vi "ChopperTEST.vi"() -> ()   [LabVIEW 2013]
uses:
  <vilib>/DAQmx/configure/timing.llb/DAQmx Timing (Sample Clock).vi
  <vilib>/DAQmx/write.llb/DAQmx Write (Digital Wfm 1Chan NSamp).vi
  <vilib>/Analysis/NI_AALBase.lvlib
  <vilib>/Analysis/1siggen.llb/Ramp Pattern by Samples.vi
  <vilib>/DAQmx/write.llb/DAQmx Write (Analog 1D Wfm NChan NSamp).vi
  <resource>/objmgr/daqmx.rc
  <vilib>/DAQmx/create/channels.llb/DAQmx Create Channel (CO-Pulse Generation-Frequency).vi
  <vilib>/DAQmx/configure/timing.llb/DAQmx Timing (Implicit).vi
  <vilib>/Waveform/DWDTOps.llb/DWDT Boolean Array to Digital.vi
  <vilib>/DAQmx/create/channels.llb/DAQmx Create Channel (AO-Voltage-Basic).vi
  <vilib>/DAQmx/create/channels.llb/DAQmx Create Channel (DO-Digital Output).vi
panel:
  in  "Source_GATE_DutyCicle (%)":dbl(slide)=4.0000000000000036 min=0.1 max=99.9 step=0.1 scale=0.0..100.0
  in  "Source_GATE_period (ms)":dbl(slide)=60.0 scale=0.0..1000.0
  out "Faraday IN 2":bool
  in  "Faraday IN":bool
  in  "Chopper ON":bool=TRUE
  out "Chopper ON 2":bool=TRUE
  in  "Vmon_L (us)":i32(slide)=920 scale=0.0..3000.0
  in  "Vmon_H (us)":i32(slide)=27 scale=0.0..1000.0
  in  "Vmon_R (us)":i32(slide)=7 scale=0.0..40.0
  in  "Vmon_min (V)":dbl=-4.0 format="%#_13g"
  in  "Vmon_max (V)":dbl format="%#_13g"
  in  "Vmon_F (us)":i32(slide)=8 scale=0.0..40.0
  in  "ACCT_F (us)":i32(slide)=10 scale=0.0..40.0
  in  "ACCT_max (V)":dbl=1.0 format="%#_13g"
  in  "ACCT_min (V)":dbl=-1.0 format="%#_13g"
  in  "ACCT_R (us)":i32(slide)=9 scale=0.0..40.0
  in  "ACCT_H (us)":i32(slide)=20 scale=0.0..1000.0
  in  "ACCT_L (us)":i32(slide)=920 scale=0.0..3000.0
  in  "CH_GATE_H (us)":i32(slide)=34 scale=0.0..100.0
  in  "CH_GATE_L (us)":i32(slide)=920 scale=0.0..3000.0
  in  "Stop Button":bool
  # "Chopper GATE (pins 65,82)"
  # "Vmon AO0 (pins 15,16)"
  # "Source GATE (pins 89,82)"
  # "ACCT AO1 (pins 31,32)"
  # "Faraday IN (pins 67,82)"
  # "Chopper ON (pins 68,82)"
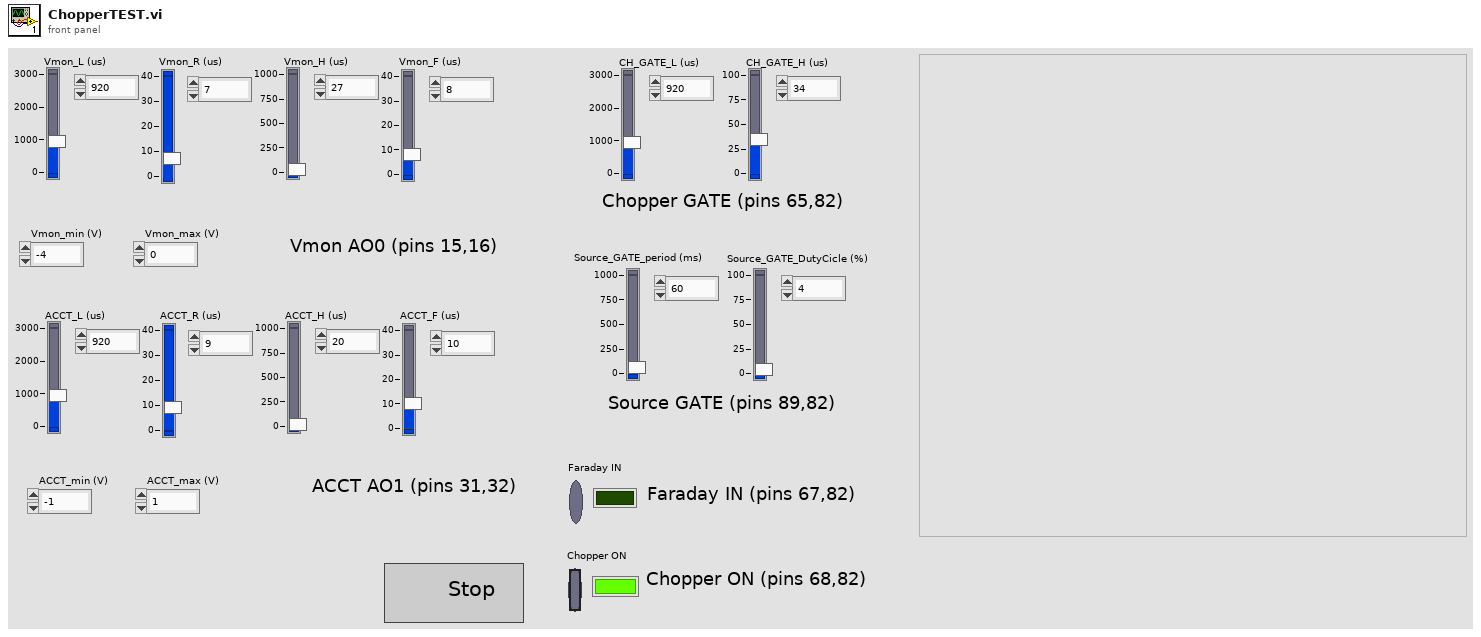
[diagram p1: front panel]
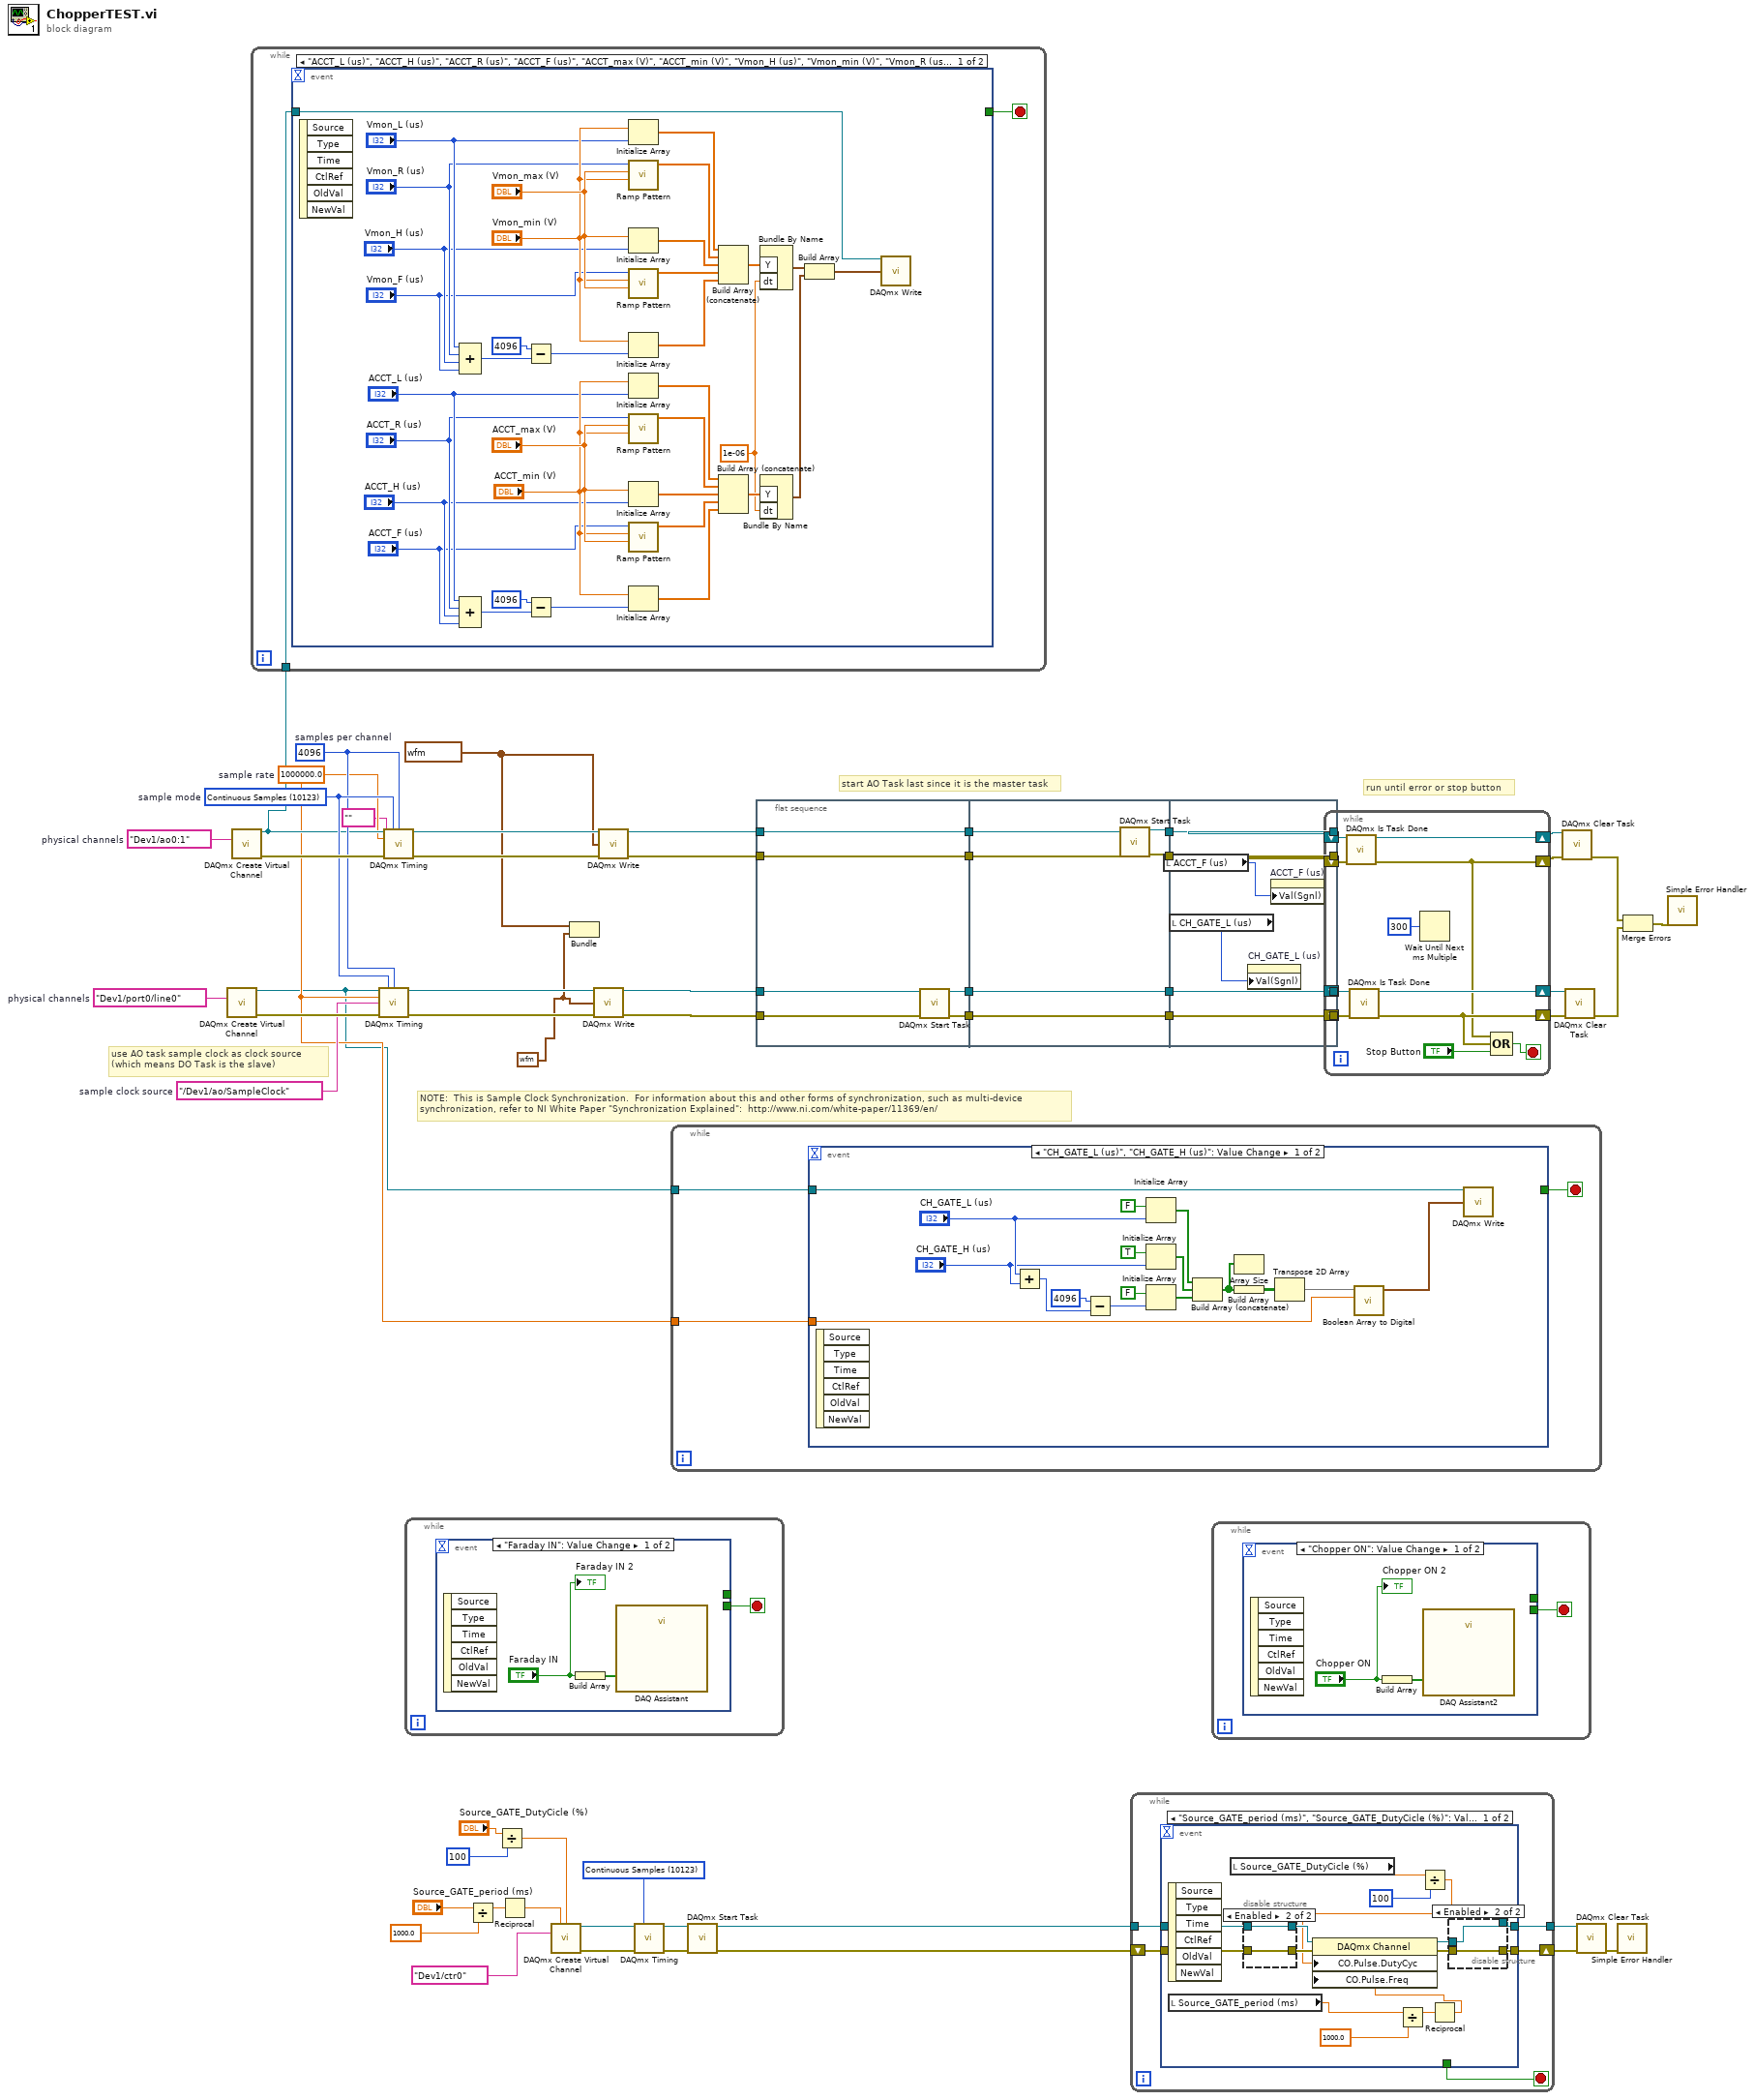
[diagram p0: block diagram]
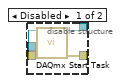
[diagram p2: hidden frame]
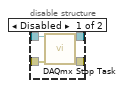
[diagram p3: hidden frame]
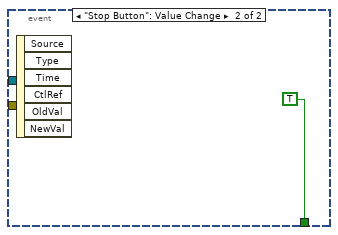
[diagram p4: hidden frame]
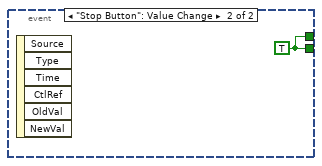
[diagram p5: hidden frame]
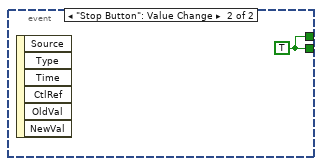
[diagram p6: hidden frame]
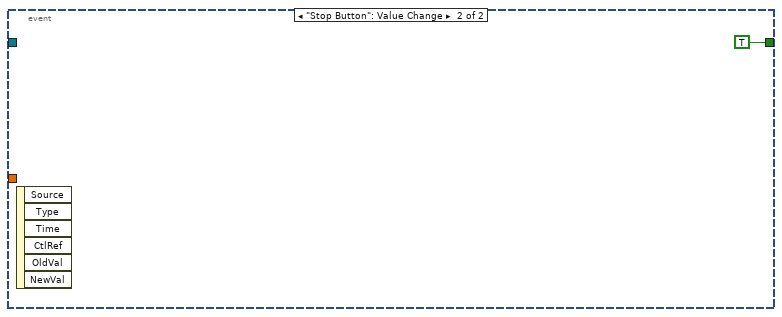
[diagram p7: hidden frame]
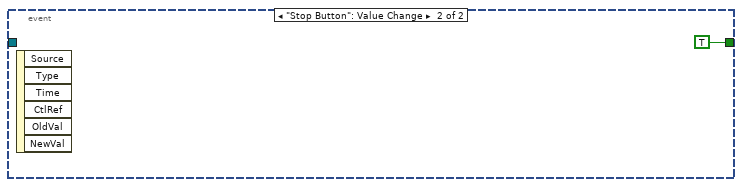
[diagram p8: hidden frame]
diagram:
  w22 = 10123 items=["Finite Samples"=10178, "Continuous Samples"=10123, "Hardware Timed Single Point"=12522] ("sample mode")
  w26 = digitalwaveform {"t0"=timestamp(0 s since 1904-01-01), "dt"=1e-06, "Y"={"transitions"=[], "data"=array4096x1[4096 elements]}} ("digital waveform 2")
  w27 = waveform(dbl)[] [{"t0"=timestamp(0 s since 1904-01-01), "dt"=1e-06, "Y"=array[4096 elements]}, {"t0"=timestamp(0 s since 1904-01-01), "dt"=1e-06, "Y"=array[4096 elements]}] ("appended array 2")
  w43 = tag "/Dev1/ao/SampleClock"  # sample clock source
  w54 = tag "Dev1/port0/line0"  # physical channels
  w44 = 4096  # samples per channel
  w45 = 10123 items=["Finite Samples"=10178, "Continuous Samples"=10123, "Hardware Timed Single Point"=12522]  # sample mode
  w25 = 1000000.0  # sample rate
  w55 = tag "Dev1/ao0:1"  # physical channels
  # "start AO Task last since it is the master task"
  # "NOTE:  This is Sample Clock Synchronization.  For information about this and other forms of synchronization, such as multi-device\nsynchronization, refer to NI White Paper \"Synchronization Explained\":  http://www.ni.com/white-paper/11369/en/"
  # "run until error or stop button"
  # "use AO task sample clock as clock source (which means DO Task is the slave)"
  n1 = call-poly <vilib>:"DAQmx Create Virtual Channel.vi"("lines"=w54) -> ("task out"=w7:refnum<k21>, "error out"=w46:errorcluster)  [unwired: 13 in]
  n2 = call-poly <vilib>:"DAQmx Create Virtual Channel.vi"("physical channels"=w55) -> ("task out"=w31:refnum<k21>, "error out"=w58:errorcluster)  [unwired: 13 in]
  n3 = while {
    tunnel: w31 -> [w60]
    stop <- w59 stop-if-true
    n4 = event shown="[0] \"ACCT_L (us)\", \"ACCT_H (us)\", \"ACCT_R (us)\", \"ACCT_F (us)\", \"ACCT_max (V)\", \"ACCT_min (V)\", \"Vmon_H (us)\", \"Vmon_min (V)\", \"Vmon_R (us)\", \"Vmon_max (V)\", \"Vmon_F (us)\", \"Vmon_L (us)\": Value Change" {
      selector: _ -> [_ _]
      dyn-events: _ -> [_ _]
      timeout: _ -> [_ _]
      tunnel: w60 -> [w86 _]
      tunnel: [_ TRUE ("Stop Button 2")] -> w59
      event "ACCT_L (us)", "ACCT_H (us)", "ACCT_R (us)", "ACCT_F (us)", "ACCT_max (V)", "ACCT_min (V)", "Vmon_H (us)", "Vmon_min (V)", "Vmon_R (us)", "Vmon_max (V)", "Vmon_F (us)", "Vmon_L (us)": Value Change {
        w64 = 1e-06 ("dt")
        n5 = event-data() -> ()  [unwired: 1 in, 6 out]
        n6 = Compound Arithmetic op=ADD("Vmon_L (us)", "Vmon_R (us)", "Vmon_H (us)", "Vmon_F (us)") -> (w66:i32)
        n7 = Compound Arithmetic op=ADD("ACCT_L (us)", "ACCT_R (us)", "ACCT_H (us)", "ACCT_F (us)") -> (w81:i32)
        n8 = Subtract(x=4096, y=w66) -> (x-y=w72:i32)
        n9 = Subtract(x=4096, y=w81) -> (x-y=w88:i32)
        n10 = Initialize Array("Vmon_min (V)", "Vmon_L (us)") -> (w79:dbl[])
        n11 = call-poly <vilib>:"Ramp Pattern.vi"("start"="Vmon_min (V)", "end"="Vmon_max (V)", "samples"="Vmon_R (us)") -> ("Ramp Pattern"=w78:dbl[])  [unwired: 7 in, 1 out]
        n12 = Initialize Array("Vmon_max (V)", "Vmon_H (us)") -> (w77:dbl[])
        n13 = call-poly <vilib>:"Ramp Pattern.vi"("start"="Vmon_max (V)", "end"="Vmon_min (V)", "samples"="Vmon_F (us)") -> ("Ramp Pattern"=w76:dbl[])  [unwired: 7 in, 1 out]
        n14 = Initialize Array("Vmon_min (V)", w72) -> (w73:dbl[])
        n15 = Initialize Array("ACCT_min (V)", "ACCT_L (us)") -> (w95:dbl[])
        n16 = call-poly <vilib>:"Ramp Pattern.vi"("start"="ACCT_min (V)", "end"="ACCT_max (V)", "samples"="ACCT_R (us)") -> ("Ramp Pattern"=w94:dbl[])  [unwired: 7 in, 1 out]
        n17 = Initialize Array("ACCT_max (V)", "ACCT_H (us)") -> (w93:dbl[])
        n18 = call-poly <vilib>:"Ramp Pattern.vi"("start"="ACCT_max (V)", "end"="ACCT_min (V)", "samples"="ACCT_F (us)") -> ("Ramp Pattern"=w92:dbl[])  [unwired: 7 in, 1 out]
        n19 = Initialize Array("ACCT_min (V)", w88) -> (w89:dbl[])
        n20 = Build Array (concatenate)(w79, w78, w77, w76, w73) -> (w65:dbl[])
        n21 = Build Array (concatenate)(w95, w94, w93, w92, w89) -> (w80:dbl[])
        n22 = Bundle By Name("Y"=w65, "dt"=w64) -> (w63:waveform(dbl))  [unwired: 1 in]
        n23 = Bundle By Name("Y"=w80, "dt"=w64) -> (w62:waveform(dbl))  [unwired: 1 in]
        n24 = Build Array(w63, w62) -> (w61:waveform(dbl)[])
        n25 = call-poly <vilib>:"DAQmx Write.vi"("task/channels in"=w86, "data"=w61) -> ()  [unwired: 11 in, 3 out]
      }
      event "Stop Button": Value Change {
        n26 = event-data() -> ()  [unwired: 1 in, 6 out]
      }
    }
  }
  n27 = call-poly <vilib>:"DAQmx Timing.vi"("task/channels in"=w7, "sample mode"=w45, "samples per channel"=w44, "rate"=w25, "source"=w43, "error in"=w46) -> ("task out"=w30:refnum<k21>, "error out"=w47:errorcluster)  [unwired: 8 in]
  n28 = call-poly <vilib>:"DAQmx Timing.vi"("task/channels in"=w31, "sample mode"=w45, "samples per channel"=w44, "rate"=w25, "source"=tag "", "error in"=w58) -> ("task out"=w42:refnum<k21>, "error out"=w41:errorcluster)  [unwired: 8 in]
  n29 = while {
    stop <- w97 stop-if-true
    n30 = event shown="[0] \"Faraday IN\": Value Change" {
      selector: _ -> [_ _]
      dyn-events: _ -> [_ _]
      timeout: _ -> [_ _]
      tunnel: [_ w100] -> _
      tunnel: [_ w100] -> w97
      event "Faraday IN": Value Change {
        n31 = event-data() -> ()  [unwired: 1 in, 6 out]
        n32 = Build Array("Faraday IN") -> (w98:bool[])
        n33 = call "DAQ Assistant"("data"=w98) -> ()  [unwired: 17 in, 2 out]
        "Faraday IN 2" <- "Faraday IN"
      }
      event "Stop Button": Value Change {
        w100 = TRUE
        n34 = event-data() -> ()  [unwired: 1 in, 6 out]
      }
    }
  }
  n35 = Divide(x="Source_GATE_period (ms)", y=1000.0) -> (x/y=w9:dbl)
  n36 = Divide(x="Source_GATE_DutyCicle (%)", y=100) -> (x/y=w11:dbl)
  n37 = Reciprocal(x=w9) -> (1/x=w8:dbl)
  n38 = call-poly <vilib>:"DAQmx Create Virtual Channel.vi"("frequency"=w8, "duty cycle"=w11, "counter"=tag "Dev1/ctr0" ("Physical Channels")) -> ("task out"=w23:refnum<k21>, "error out"=w24:errorcluster)  [unwired: 6 in, 5 out]
  n39 = Bundle("appended array 2"=w27, "digital waveform 2"=w26) -> ()  [unwired: 1 in, 1 out]
  n40 = call-poly <vilib>:"DAQmx Write.vi"("task/channels in"=w30, "data"=w26, "error in"=w47) -> ("task out"=w48:refnum<k21>, "error out"=w49:errorcluster)  [unwired: 10 in, 1 out]
  n41 = call-poly <vilib>:"DAQmx Write.vi"("task/channels in"=w42, "data"=w27, "error in"=w41) -> ("task out"=w38:refnum<k21>, "error out"=w37:errorcluster)  [unwired: 10 in, 1 out]
  n42 = call-poly <vilib>:"DAQmx Timing.vi"("task/channels in"=w23, "sample mode"=w22, "error in"=w24) -> ("task out"=w20:refnum<k21>, "error out"=w21:errorcluster)  [unwired: 11 in]
  n43 = while {
    tunnel: w25 -> [w103]
    tunnel: w7 -> [w102]
    stop <- w101 stop-if-true
    n44 = event shown="[0] \"CH_GATE_L (us)\", \"CH_GATE_H (us)\": Value Change" {
      selector: _ -> [_ _]
      dyn-events: _ -> [_ _]
      timeout: _ -> [_ _]
      tunnel: w103 -> [w114 _]
      tunnel: w102 -> [w105 _]
      tunnel: [_ TRUE ("Stop Button 3")] -> w101
      event "CH_GATE_L (us)", "CH_GATE_H (us)": Value Change {
        n45 = event-data() -> ()  [unwired: 1 in, 6 out]
        n46 = Add(x="CH_GATE_L (us)", y="CH_GATE_H (us)") -> (x+y=w108:i32)
        n47 = Subtract(x=4096, y=w108) -> (x-y=w106:i32)
        n48 = Initialize Array(FALSE, "CH_GATE_L (us)") -> (w118:bool[])
        n49 = Initialize Array(TRUE, "CH_GATE_H (us)") -> (w117:bool[])
        n50 = Initialize Array(FALSE, w106) -> (w110:bool[])
        n51 = Build Array (concatenate)(w118, w117, w110) -> (w115:bool[])
        n52 = Array Size(array=w115) -> ()  [unwired: 1 out]
        n53 = Build Array(w115) -> (w116:bool[][])
        n54 = Transpose 2D Array(2D array=w116) -> (transposed array=w113:bool[][])
        n55 = call-poly <vilib>:"Boolean Array to Digital.vi"("sample rate"=w114, "boolean array"=w113) -> ("digital waveform"=w104:digitalwaveform)  [unwired: 8 in, 1 out]
        n56 = call-poly <vilib>:"DAQmx Write.vi"("task/channels in"=w105, "data"=w104) -> ()  [unwired: 11 in, 3 out]
      }
      event "Stop Button": Value Change {
        n57 = event-data() -> ()  [unwired: 1 in, 6 out]
      }
    }
  }
  n58 = call <vilib>:"DAQmx Start Task.vi"("task/channels in"=w20, "error in"=w21) -> ("task out"=w15:refnum<k21>, "error out"=w16:errorcluster)  [unwired: 12 out]
  n59 = flat-sequence {
    tunnel: w49 -> [w125]
    tunnel: w48 -> [w124]
    tunnel: [w127] -> w40
    tunnel: [w126] -> w39
    tunnel: w38 -> [w123]
    tunnel: w37 -> [w122]
    tunnel: [w123] -> w29
    tunnel: [w122] -> w28
    tunnel: w40 -> [w133]
    tunnel: w39 -> [w132]
    tunnel: w29 -> [w131]
    tunnel: w28 -> [w130]
    tunnel: [w133] -> w4
    tunnel: [w132] -> w3
    tunnel: [w129] -> w2
    tunnel: [w128] -> w1
    tunnel: [w136] -> w35
    tunnel: [w137] -> w36
    tunnel: [w138] -> w50
    tunnel: [w139] -> w51
    tunnel: w4 -> [w139]
    tunnel: w3 -> [w138]
    tunnel: w2 -> [w137]
    tunnel: w1 -> [w136]
    frame #0 {
      n60 = call <vilib>:"DAQmx Start Task.vi"("task/channels in"=w124, "error in"=w125) -> ("task out"=w126:refnum<k21>, "error out"=w127:errorcluster)  [unwired: 12 in]
    }
    frame #1 {
      n61 = call <vilib>:"DAQmx Start Task.vi"("task/channels in"=w131, "error in"=w130) -> ("task out"=w129:refnum<k21>, "error out"=w128:errorcluster)  [unwired: 12 in]
    }
    frame #2 {
      n62 = local read "ACCT_F (us)"() -> (w134:i32)
      n63 = local read "CH_GATE_L (us)"() -> (w135:i32)
      n64 = property on="CH_GATE_L (us)" class="Slide (strict)"("Val(Sgnl)"=w135) -> ()  [unwired: 2 in, 2 out]
      n65 = property on="ACCT_F (us)" class="Slide (strict)"("Val(Sgnl)"=w134) -> ()  [unwired: 2 in, 2 out]
    }
  }
  n66 = while {
    tunnel: w15 -> [w144]
    tunnel: [w143] -> w17
    shift-right: [w142] -> w18
    shift-left: w16 -> [w141]
    stop <- w140 stop-if-true
    n67 = event shown="[0] \"Source_GATE_period (ms)\", \"Source_GATE_DutyCicle (%)\": Value Change" {
      selector: _ -> [_ _]
      dyn-events: _ -> [_ _]
      timeout: _ -> [_ _]
      tunnel: w144 -> [w159 _]
      tunnel: [w149 _] -> w143
      tunnel: [w158 _] -> w142
      tunnel: w141 -> [w157 _]
      tunnel: [_ TRUE] -> w140
      event "Source_GATE_period (ms)", "Source_GATE_DutyCicle (%)": Value Change {
        n68 = event-data() -> ()  [unwired: 1 in, 6 out]
        n69 = local read "Source_GATE_period (ms)"() -> (w146:dbl)
        n70 = local read "Source_GATE_DutyCicle (%)"() -> (w152:dbl)
        n71 = disable-structure shown="Enabled" {
          disable-tunnel: w159 -> [w169 w171]
          disable-tunnel: w157 -> [w168 w170]
          disable-tunnel: [w167 w171] -> w156
          disable-tunnel: [w166 w170] -> w154
          frame Disabled {
            n72 = call <vilib>:"DAQmx Stop Task.vi"("task/channels in"=w169, "error in"=w168) -> ("task out"=w167:refnum<k21>, "error out"=w166:errorcluster)  [unwired: 12 out]
          }
          frame Enabled {
          }
        }
        n73 = Divide(x=w146, y=1000.0) -> (x/y=w147:dbl)
        n74 = Divide(x=w152, y=100) -> (x/y=w150:dbl)
        n75 = Reciprocal(x=w147) -> (1/x=w145:dbl)
        n76 = property class="DAQmx Channel"(reference=w156, error in=w154, "CO.Pulse.DutyCyc"=w150, "CO.Pulse.Freq"=w145) -> (reference out=w155:refnum<k21>, error out=w153:errorcluster)
        n77 = disable-structure shown="Enabled" {
          disable-tunnel: [w162 w164] -> w158
          disable-tunnel: w155 -> [w161 w165]
          disable-tunnel: w153 -> [w160 w164]
          disable-tunnel: [w163 w165] -> w149
          frame Disabled {
            n78 = call <vilib>:"DAQmx Start Task.vi"("task/channels in"=w161, "error in"=w160) -> ("task out"=w163:refnum<k21>, "error out"=w162:errorcluster)  [unwired: 12 out]
          }
          frame Enabled {
          }
        }
      }
      event "Stop Button": Value Change {
        n79 = event-data() -> ()  [unwired: 1 in, 6 out]
      }
    }
  }
  n80 = while {
    stop <- w173 stop-if-true
    n81 = event shown="[0] \"Chopper ON\": Value Change" {
      selector: _ -> [_ _]
      dyn-events: _ -> [_ _]
      timeout: _ -> [_ _]
      tunnel: [_ w176] -> _
      tunnel: [_ w176] -> w173
      event "Chopper ON": Value Change {
        n82 = event-data() -> ()  [unwired: 1 in, 6 out]
        n83 = Build Array("Chopper ON") -> (w174:bool[])
        n84 = call "DAQ Assistant2"("data"=w174) -> ()  [unwired: 17 in, 2 out]
        "Chopper ON 2" <- "Chopper ON"
      }
      event "Stop Button": Value Change {
        w176 = TRUE
        n85 = event-data() -> ()  [unwired: 1 in, 6 out]
      }
    }
  }
  n86 = while {
    shift-right: [w180] -> w53
    shift-left: w51 -> [w185]
    shift-right: [w186] -> w52
    shift-left: w50 -> [w184]
    shift-right: [w187] -> w57
    shift-left: w36 -> [w183]
    shift-right: [w179] -> w56
    shift-left: w35 -> [w182]
    stop <- w178 stop-if-true
    n87 = call <vilib>:"DAQmx Is Task Done.vi"("task/channels in"=w183, "error in"=w182) -> ("task out"=w187:refnum<k21>, "error out"=w179:errorcluster)  [unwired: 11 in, 1 out]
    n88 = call <vilib>:"DAQmx Is Task Done.vi"("task/channels in"=w184, "error in"=w185) -> ("task out"=w186:refnum<k21>, "error out"=w180:errorcluster)  [unwired: 11 in, 1 out]
    n89 = Wait Until Next ms Multiple(millisecond multiple=u32 300) -> ()  [unwired: 1 out]
    n90 = Compound Arithmetic op=OR(w179, w180, "Stop Button") -> (w178:bool)
  }
  n91 = call <vilib>:"DAQmx Clear Task.vi"("task in"=w57, "error in"=w56) -> ("error out"=w33:errorcluster)  [unwired: 13 in]
  n92 = call <vilib>:"DAQmx Clear Task.vi"("task in"=w52, "error in"=w53) -> ("error out"=w32:errorcluster)  [unwired: 13 in]
  n93 = call <vilib>:"DAQmx Clear Task.vi"("task in"=w17, "error in"=w18) -> ("error out"=w19:errorcluster)  [unwired: 13 out]
  n94 = call <vilib>:"Simple Error Handler.vi"("error in (no error)"=w19) -> ()  [unwired: 4 in, 5 out]
  n95 = Merge Errors(w33, w32) -> (w34:errorcluster)
  n96 = call <vilib>:"Simple Error Handler.vi"("error in (no error)"=w34) -> ()  [unwired: 4 in, 5 out]
